vi "Alarm_Control.vi"(0 "State":T1, 3 "error in":errorcluster caption="错误输入（无错误）") -> (1 "DO0 Software":bool, 2 "DO1 Software":bool, 4 "error out":errorcluster caption="错误输出")   [LabVIEW 2020]
uses:
  Controls/State.ctl
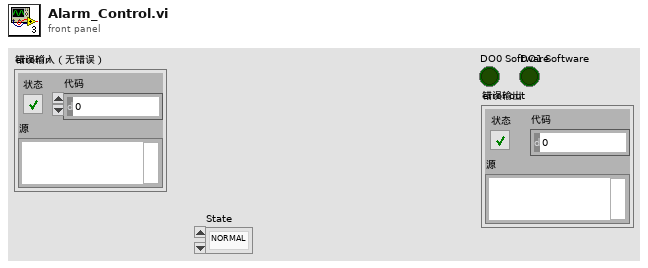
[diagram p1: front panel]
types:
  T1 = typedef "State.ctl" = enum16{"NORMAL", "SUSPECT", "COUNTDOWN", "ALARM", "RESET"}
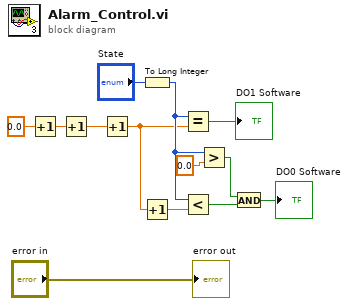
[diagram p0: block diagram]
diagram:
  n1 = Increment(x=0.0) -> (x+1=w5:dbl)
  n2 = Increment(x=w5) -> (x+1=w4:dbl)
  n3 = Increment(x=w4) -> (x+1=w3:dbl)
  n4 = To Long Integer(number="State") -> (32bit integer=w8:i32)
  n5 = Increment(x=w3) -> (x+1=w2:dbl)
  n6 = Equal?(x=w8, y=w3) -> (x = y?=→"DO1 Software":bool)
  n7 = Less?(x=w8, y=w2) -> (x < y?=w6:bool)
  n8 = Greater?(x=w8, y=0.0) -> (0:w7:bool)
  n9 = And(x=w7, y=w6) -> (x .and. y?=→"DO0 Software":bool)
  "error out" <- "error in"
